vi "proxy_for_client_plugin.vi"(10 "Config":string, 11 "file path (use dialog)":path=path "C:/DEV/emea-tra-iPerf_bus_load_test/support/iperf_proxies/iperf_proxies/iperf_client.json") -> ()   [LabVIEW 2026]
doc: "Demonstrates the use of the OS IP Stack TCP functions to connect to a TCP server VI and receive data, via a proxy server running within the XNET IP Stack."
panel:
  in  "stop":bool
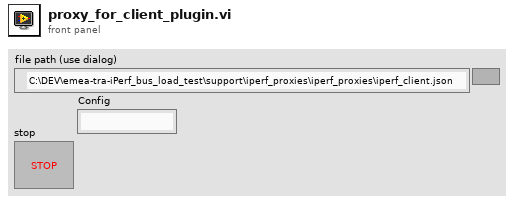
[diagram p1: front panel]
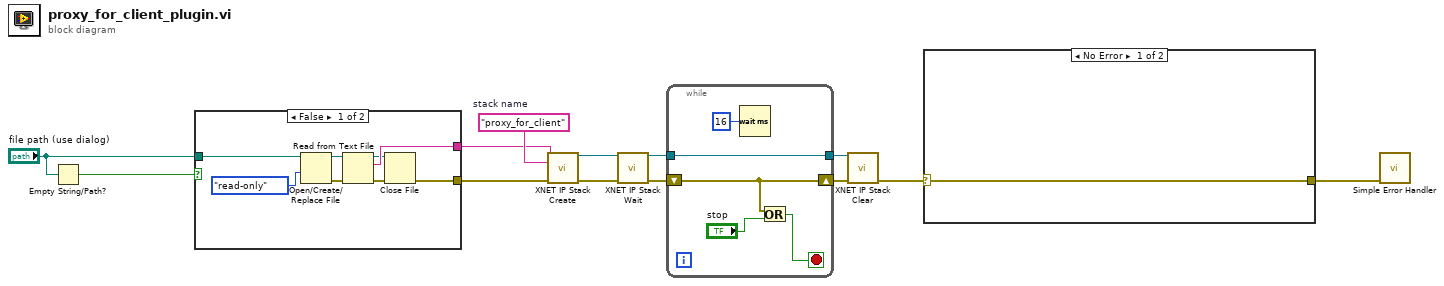
[diagram p0: block diagram]
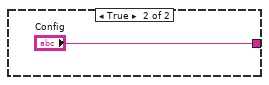
[diagram p2: hidden frame]
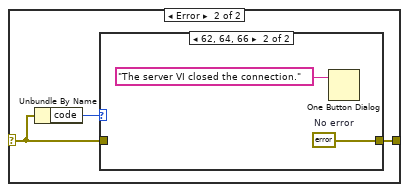
[diagram p3: hidden frame]
diagram:
  w9 = "proxy_for_client"  # stack name
  n1 = Empty String/Path?(string/path="file path (use dialog)") -> (empty?=w1:bool)
  n2 = case shown="False" w1 {
    tunnel: "file path (use dialog)" -> [w21 _]
    tunnel: [w17 "Config"] -> w4
    tunnel: [w14 _] -> w3
    frame False {
      n3 = Open/Create/Replace File(file path (use dialog)=w21, access (0:read/write)=enum16{"read/write", "read-only", "write-only"}."read-only") -> (refnum out=w19:refnum<file>, error out=w18:errorcluster)  [unwired: 4 in, 1 out]
      n4 = Read from Text File(file (use dialog)=w19, error in=w18) -> (refnum out=w16:refnum<file>, text=w17:string, error out=w15:errorcluster)  [unwired: 2 in, 1 out]
      n5 = Close File(refnum=w16, error in=w15) -> (error out=w14:errorcluster)  [unwired: 1 out]
    }
    frame True {
    }
  }
  n6 = call <vilib>:"XNET IP Stack Create.vi"("config"=w4, "stack name"=w9, "error in"=w3) -> ("stack out"=w12:refnum<k21>, "error out"=w13:errorcluster)  [unwired: 11 in]
  n7 = call <vilib>:"XNET IP Stack Wait.vi"("stack in"=w12, "error in"=w13) -> ("stack out"=w6:refnum<k21>, "error out"=w7:errorcluster)  [unwired: 12 in]
  n8 = while {
    shift-right: [w27] -> w8
    shift-left: w7 -> [w27]
    tunnel: w6 -> [w24]
    tunnel: [w24] -> w5
    stop <- w25 stop-if-true
    n9 = Wait (ms)(milliseconds to wait=u32 16) -> ()  [unwired: 1 out]
    n10 = Or(x=w27, y="stop") -> (x .or. y?=w25:bool)
  }
  n11 = call <vilib>:"XNET IP Stack Clear.vi"("stack"=w5, "error in"=w8) -> ("error out"=w11:errorcluster)  [unwired: 13 in]
  n12 = case shown="No Error" w11 {
    selector: w11 -> [w28 w30]
    tunnel: [w28 w29] -> w10
    frame No Error {
    }
    frame Error {
      n13 = Unbundle By Name(w30) -> ("code"=w31:i32)
      n14 = case shown="62, 64, 66" w31 {
        tunnel: w30 -> [w32 _]
        tunnel: [w32 w34] -> w29
        frame Default {
        }
        frame 62, 64, 66 {
          w34 = errorcluster {"status"=FALSE, "code"=0, "source"=""}  # No error
          n15 = One Button Dialog(message="The server VI closed the connection." ("Server Closed")) -> ()  [unwired: 1 in, 1 out]
        }
      }
    }
  }
  n16 = call <vilib>:"Simple Error Handler.vi"("error in (no error)"=w10) -> ()  [unwired: 4 in, 5 out]
